vi "Main.vi"() -> ()   [LabVIEW 2020]
doc: "Gold Hunter. Start: App_Init (queues, notifier), Game_Start (world, highscores), sprites, HUD and title pictures, Window_Setup, Audio_Start. Main (same as caller) holds the loops for keys (Key Down / Key Up by ScanCode and the Stop button -> Key_Send -> queue) and picture (Render_Frame in its own system -> Screen). Game_Loop (standard: Engine_Tick 60 times per second, Frame_Pace) and Sound_Loop (other 2: Audio_Block) are subVIs with their own loop. Timing log of ticks and frames to Resourcesòta, only when the cheat mode was used. Drag the window by its top border (mouse). End: Esc on the title screen, a click on the X at the top right of the screen, Stop, or Panel Close? (discarded) - the game ends normally, then Main closes its window. Keys: arrows = walk, climb, choose letters; Space = jump; Enter = start; Esc/P = pause; Z U L U = cheat (all rooms lit, endless lives)."
uses:
  Source/App/GH_App.lvlib
  Source/Engine/GH_Engine.lvlib
  Source/Render/GH_Render.lvlib
panel:
  out "error out":errorcluster
  in  "Sound":bool=TRUE
  out "FPS":dbl
  out "Screen":picture
  in  "Stop":bool
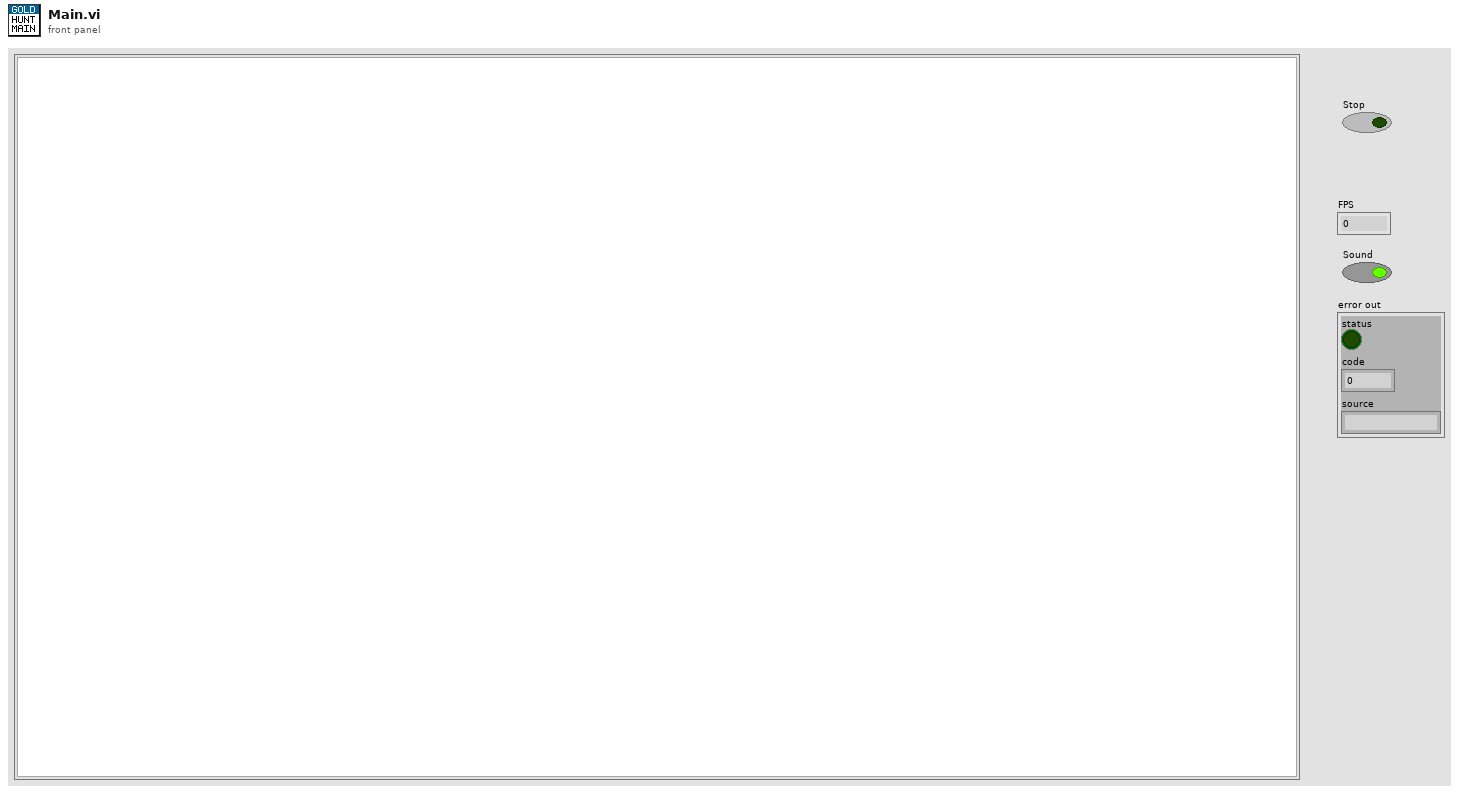
[diagram p1: front panel]
types:
  T1 = cluster{"RoomKey":i32, "Key":i32, "NameKey":i32, "Lit":u8[][], "Dim":u8[][], "Dark":u8[][], "Comp":u8[][], "Template":cluster{"image type":i32, "image depth":i32, "image":u8[], "mask":u8[], "colors":u32[], "Rectangle":cluster{"left":i16, "top":i16, "right":i16, "bottom":i16}}, "CX":i32, "CY":i32, "X1":i32, "Y1":i32, "X2":i32, "Y2":i32, "Prev":cluster{"Kind":i32, "X10":i32, "Y10":i32, "Dir":i32, "Mode":i32}[], "HudKey":i32, "HudScore":i32, "HudTime":i32, "Full":cluster{"image type":i32, "image depth":i32, "image":u8[], "mask":u8[], "colors":u32[], "Rectangle":cluster{"left":i16, "top":i16, "right":i16, "bottom":i16}}[]}
  T2 = cluster{"Keys":refnum<queue>, "Frames":refnum<notifier>, "Sounds":refnum<queue>}
  T3 = cluster{"Tick":u32, "Phase":i32, "PhaseTicks":i32, "Level":i32, "Room":i32, "X10":i32, "Y10":i32, "VY10":i32, "Mode":i32, "Facing":i32, "Run":i32, "Vert":i32, "StandY":i32, "EntryX10":i32, "EntryY10":i32, "EntryMode":i32, "Lives":i32, "Score":i32, "NextLife":i32, "KeyR":i32, "KeyB":i32, "KeyY":i32, "Torch":bool, "FloorPhase":i32, "Dead":bool, "LevelStart":bool, "Quit":bool, "Sound":i32, "Seed":u32, "DemoStep":i32, "Tiles":u8[][], "World":cluster{"ID":string, "Depth":i32, "Column":i32, "Tiles":u8[][]}[], "Enemies":cluster{"Kind":i32, "X10":i32, "Y10":i32, "Dir":i32, "Mode":i32}[], "Highscores":cluster{"Score":i32, "Name":string}[], "Name":i32[], "Cursor":i32}
  T4 = cluster{"ID":string, "Depth":i32, "Column":i32, "Tiles":u8[][]}[]
  T5 = cluster{"image type":i32, "image depth":i32, "image":u8[], "mask":u8[], "colors":u32[], "Rectangle":cluster{"left":i16, "top":i16, "right":i16, "bottom":i16}}
  T6 = typedef "LVPoint32TypeDef.ctl" = cluster{"Horizontal":i32, "Vertical":i32}
  T7 = cluster{"Current":dbl[], "Position":i32, "Priority":i32, "Music":bool, "MusicPos":i32}
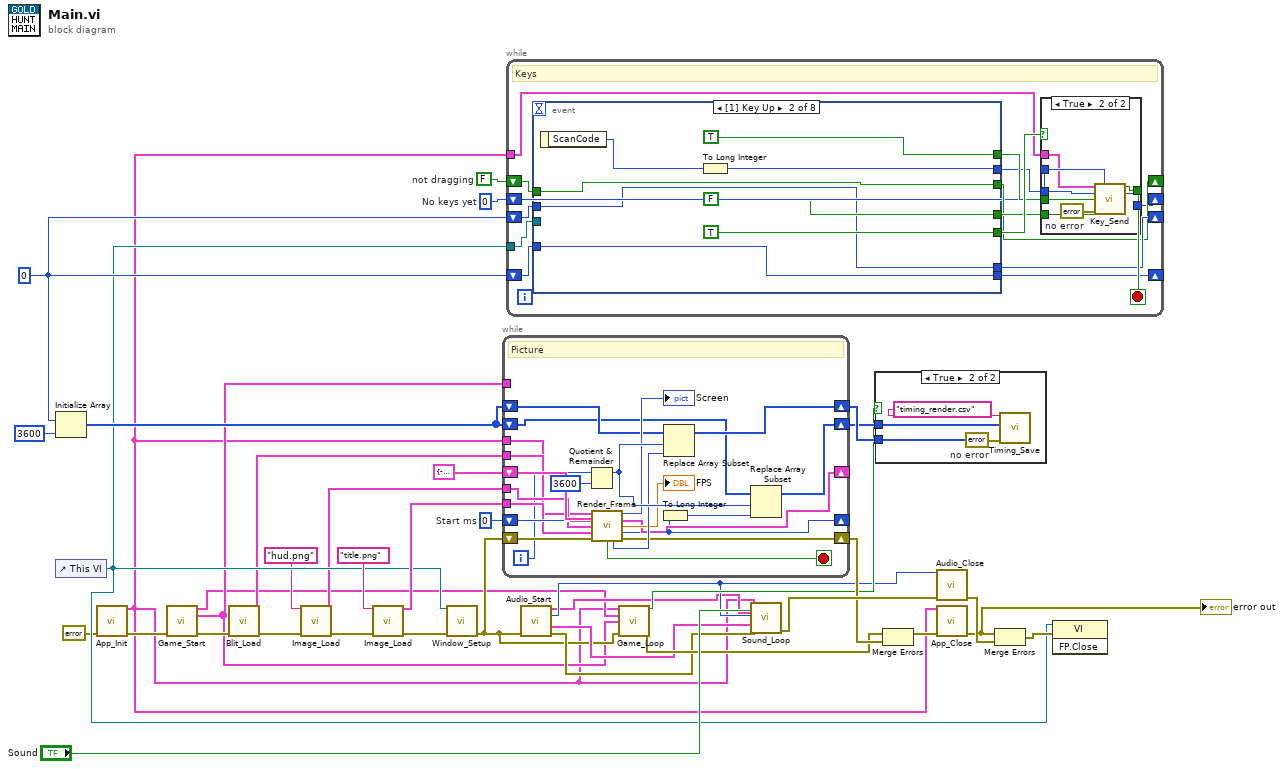
[diagram p0: block diagram]
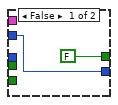
[diagram p3: hidden frame]
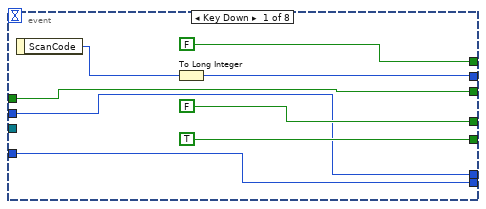
[diagram p4: hidden frame]
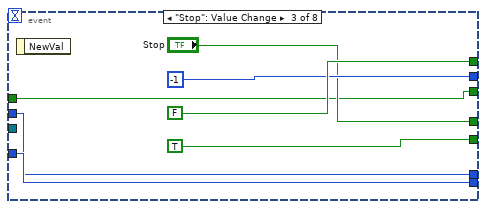
[diagram p5: hidden frame]
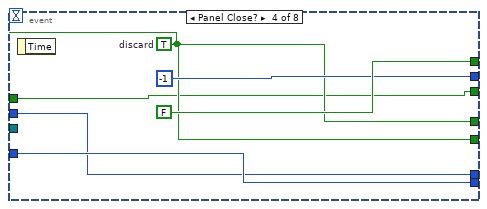
[diagram p6: hidden frame]
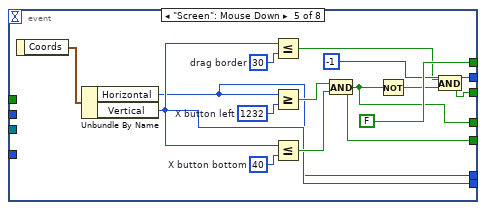
[diagram p7: hidden frame]
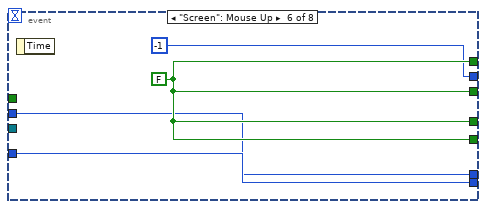
[diagram p8: hidden frame]
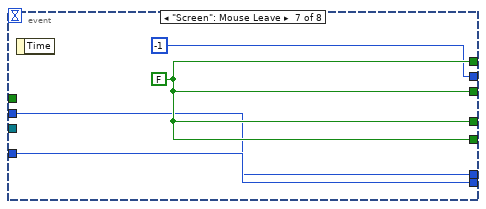
[diagram p9: hidden frame]
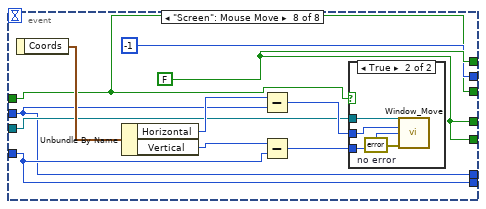
[diagram p10: hidden frame]
diagram:
  w27 = FALSE  # not dragging
  w24 = 0
  w23 = 0  # No keys yet
  w22 = u32 0  # Start ms
  n1 = Initialize Array(w24, 3600) -> (w26:i32[])
  n2 = control-ref of="This VI"() -> (w12:refnum<vi>)
  n3 = call "App_Init.vi"("error in"=errorcluster {"status"=FALSE, "code"=0, "source"=""} ("no error")) -> ("Channels"=w2:T2, "error out"=w3:errorcluster)  [unwired: 13 in]
  n4 = call "Game_Start.vi"("error in"=w3) -> ("State"=w4:T3, "Rooms"=w5:T4, "error out"=w6:errorcluster)  [unwired: 12 in]
  n5 = call "Blit_Load.vi"("error in"=w6) -> ("Sprites"=w7:cluster{"Pix":u8[][], "Mask":u8[][]}[], "error out"=w8:errorcluster)  [unwired: 13 in]
  n6 = call "Image_Load.vi"("File name"="hud.png" ("HUD file"), "error in"=w8) -> ("Image"=w10:T5, "error out"=w11:errorcluster)  [unwired: 12 in]
  n7 = call "Image_Load.vi"("File name"="title.png" ("Title file"), "error in"=w11) -> ("Image"=w14:T5, "error out"=w15:errorcluster)  [unwired: 12 in]
  n8 = call "Window_Setup.vi"("VI"=w12, "error in"=w15) -> ("error out"=w16:errorcluster)  [unwired: 13 in]
  n9 = while {
    shift-right: [w45] -> _
    shift-left: w22 -> [w44]
    shift-right: [w49] -> _
    shift-left: T1 {"RoomKey"=-1, "Key"=-1, "NameKey"=-1, "Lit"=[], "Dim"=[], "Dark"=[], "Comp"=[], "Template"={"image type"=0, "image depth"=0, "image"=[], "mask"=[], "colors"=[], "Rectangle"={"left"=0, "top"=0, "right"=0, "bottom"=0}}, "CX"=-1, "CY"=-1, "X1"=0, "Y1"=0, "X2"=0, "Y2"=0, "Prev"=[], "HudKey"=-1, "HudScore"=-1, "HudTime"=-1, "Full"=[]} ("Nothing drawn yet") -> [w48]
    tunnel: w2 -> [w40]
    shift-right: [w51] -> w31
    shift-left: w26 -> [w50]
    shift-right: [w53] -> w32
    shift-left: w26 -> [w52]
    tunnel: w5 -> [_]
    tunnel: w7 -> [w41]
    tunnel: w10 -> [w42]
    tunnel: w14 -> [w43]
    shift-right: [w47] -> w30
    shift-left: w16 -> [w46]
    i -> [w39]
    stop <- w56 stop-if-true
    # "Picture"
    n10 = Quotient & Remainder(x=w39, y=3600) -> (x-y*floor(x/y)=w59:i32)  [unwired: 1 out]
    n11 = call "Render_Frame.vi"("Channels"=w40, "Memory"=w48, "Last ms"=w44, "Sprites"=w41, "Hud"=w42, "Title"=w43, "error in"=w46) -> ("Picture"=→"Screen":picture, "Memory out"=w49:T1, "FPS"=→"FPS":dbl, "Now ms"=w45:u32, "Stop"=w56:bool, "Tick"=w57:i32, "error out"=w47:errorcluster)  [unwired: 2 in]
    n12 = To Long Integer(number=w45) -> (32bit integer=w60:i32)
    n13 = Replace Array Subset(array=w52, new element=w57, index=w59) -> (w53:i32[])
    n14 = Replace Array Subset(array=w50, new element=w60, index=w59) -> (w51:i32[])
  }
  n15 = while {
    shift-right: [w64] -> _
    shift-left: w23 -> [w63]
    shift-right: [w66] -> _
    shift-left: w27 -> [w65]
    shift-right: [w68] -> _
    shift-left: w24 -> [w67]
    shift-right: [w70] -> _
    shift-left: w24 -> [w69]
    tunnel: w2 -> [w61]
    tunnel: w12 -> [w62]
    stop <- w75 stop-if-true
    # "Keys"
    n16 = event shown="[1] Key Up" {
      selector: _ -> [_ _ _ _ _ _ _ _]
      dyn-events: _ -> [_ _ _ _ _ _ _ _]
      timeout: _ -> [_ _ _ _ _ _ _ _]
      tunnel: [FALSE TRUE FALSE FALSE FALSE w132 w136 w147] -> w72
      tunnel: [FALSE FALSE "Stop" w112 w122 w132 w136 w147] -> w73
      tunnel: [TRUE TRUE TRUE w112 w122 w132 w136 w147] -> w74
      tunnel: w65 -> [w86 w94 w102 w109 _ _ _ w137]
      tunnel: w67 -> [w87 w95 w103 w110 _ w129 w133 w138]
      tunnel: w69 -> [w88 w96 w104 w111 _ w130 w134 w139]
      tunnel: w62 -> [_ _ _ _ _ _ _ w140]
      tunnel: [w90 w98 -1 -1 -1 -1 -1 -1] -> w71
      tunnel: [w86 w94 w102 w109 w126 w132 w136 w137] -> w66
      tunnel: [w87 w95 w103 w110 w116 w129 w133 w138] -> w68
      tunnel: [w88 w96 w104 w111 w117 w130 w134 w139] -> w70
      event Key Down {
        n17 = event-data() -> ("ScanCode"=w89:i16)  [unwired: 1 in]
        n18 = To Long Integer(number=w89) -> (32bit integer=w90:i32)
      }
      event Key Up {
        n19 = event-data() -> ("ScanCode"=w97:i16)  [unwired: 1 in]
        n20 = To Long Integer(number=w97) -> (32bit integer=w98:i32)
      }
      event "Stop": Value Change {
        n21 = event-data() -> ()  [unwired: 1 in, 1 out]
      }
      event Panel Close? {
        w112 = TRUE  # discard
        n22 = event-data("Discard?"=w112) -> ()  [unwired: 1 in, 1 out]
        n23 = event-data() -> ()  [unwired: 1 in, 1 out]
      }
      event "Screen": Mouse Down {
        w123 = 30  # drag border
        w120 = 40  # X button bottom
        w118 = 1232  # X button left
        n24 = event-data() -> ("Coords"=w115:T6)  [unwired: 1 in]
        n25 = Unbundle By Name(w115) -> ("Horizontal"=w116:i32, "Vertical"=w117:i32)
        n26 = Less Or Equal?(x=w117, y=w123) -> (x <= y?=w124:bool)
        n27 = Greater Or Equal?(x=w116, y=w118) -> (x >= y?=w119:bool)
        n28 = Less Or Equal?(x=w117, y=w120) -> (x <= y?=w121:bool)
        n29 = And(x=w119, y=w121) -> (x .and. y?=w122:bool)
        n30 = Not(x=w122) -> (.not. x?=w125:bool)
        n31 = And(x=w124, y=w125) -> (x .and. y?=w126:bool)
      }
      event "Screen": Mouse Up {
        w132 = FALSE
        n32 = event-data() -> ()  [unwired: 1 in, 1 out]
      }
      event "Screen": Mouse Leave {
        w136 = FALSE
        n33 = event-data() -> ()  [unwired: 1 in, 1 out]
      }
      event "Screen": Mouse Move {
        w147 = FALSE
        n34 = event-data() -> ("Coords"=w141:T6)  [unwired: 1 in]
        n35 = Unbundle By Name(w141) -> ("Horizontal"=w142:i32, "Vertical"=w143:i32)
        n36 = Subtract(x=w142, y=w138) -> (x-y=w144:i32)
        n37 = Subtract(x=w143, y=w139) -> (x-y=w145:i32)
        n38 = case shown="True" w137 {
          tunnel: w140 -> [_ w148]
          tunnel: w144 -> [_ w149]
          tunnel: w145 -> [_ w150]
          frame False {
          }
          frame True {
            w151 = errorcluster {"status"=FALSE, "code"=0, "source"=""}  # no error
            n39 = call "Window_Move.vi"("VI"=w148, "DX"=w149, "DY"=w150, "error in"=w151) -> ()  [unwired: 11 in, 1 out]
          }
        }
      }
    }
    n40 = case shown="True" w74 {
      tunnel: w72 -> [_ w80]
      tunnel: w73 -> [_ w81]
      tunnel: w63 -> [w76 w82]
      tunnel: w61 -> [_ w78]
      tunnel: w71 -> [_ w79]
      tunnel: [FALSE w84] -> w75
      tunnel: [w76 w85] -> w64
      frame False {
      }
      frame True {
        w83 = errorcluster {"status"=FALSE, "code"=0, "source"=""}  # no error
        n41 = call "Key_Send.vi"("Channels"=w78, "History"=w82, "ScanCode"=w79, "Released"=w80, "Quit"=w81, "error in"=w83) -> ("Quit out"=w84:bool, "History out"=w85:i32)  [unwired: 7 in, 1 out]
      }
    }
  }
  n42 = call "Audio_Start.vi"("error in"=w16) -> ("Bank"=w17:cluster{"Y":dbl[]}[], "Task ID"=w18:u32, "Mixer"=w19:T7, "error out"=w20:errorcluster)  [unwired: 11 in]
  n43 = call "Game_Loop.vi"("Channels"=w2, "State"=w4, "Rooms"=w5, "error in"=w16) -> ("Cheat used"=w28:bool, "error out"=w29:errorcluster)  [unwired: 10 in]
  n44 = call "Sound_Loop.vi"("Channels"=w2, "Sound"="Sound", "Bank"=w17, "Task ID"=w18, "Mixer"=w19, "error in"=w20) -> ("error out"=w34:errorcluster)  [unwired: 9 in]
  n45 = case shown="True" w28 {
    tunnel: w31 -> [_ w152]
    tunnel: w32 -> [_ w153]
    frame False {
    }
    frame True {
      w155 = errorcluster {"status"=FALSE, "code"=0, "source"=""}  # no error
      n46 = call "Timing_Save.vi"("File name"="timing_render.csv", "Ms"=w152, "Tick"=w153, "error in"=w155) -> ()  [unwired: 11 in, 1 out]
    }
  }
  n47 = Merge Errors(w29, w30) -> (w35:errorcluster)
  n48 = call "Audio_Close.vi"("Task ID"=w18, "error in"=w34) -> ("error out"=w37:errorcluster)  [unwired: 13 in]
  n49 = call "App_Close.vi"("Channels"=w2, "error in"=w35) -> ("error out"=w36:errorcluster)  [unwired: 13 in]
  "error out" <- w36
  n50 = Merge Errors(w36, w37) -> (w38:errorcluster)
  n51 = invoke class="VI" method="FP.Close"(reference=w12, error in=w38) -> ()  [unwired: 1 in, 3 out]
